vi "Compile and Export Settings.vi"(8 "error in (no error)":errorcluster, 11 "Device Item Ref in":T1 format="%.0x") -> (0 "error out":errorcluster)   [LabVIEW 2015, in "Protection and Counter Addon System Explorer.lvlib"]
uses:
  Protection and Counter Addon System Explorer.lvlib
  <vilib>/NI Veristand/Custom Device API/Custom Device Item Ref.ctl
  Shared/Types/Exported.OnCompile.ctl
  Shared/Types/XNET Settings.ctl
  SubModules/Frame Protection Support/Source/Shared/Types/Exported Frame Settings.ctl
  SubModules/Frame Protection Support/Source/Shared/Types/Exported Frame Type.ctl
  SubModules/Frame Protection Support/Source/Shared/Types/Exported Protection Settings.ctl
  SubModules/Frame Protection Support/Source/Shared/Types/Protection Type.ctl
  SubModules/Frame Protection Support/Source/Shared/Types/XNET Signal Configuration.ctl
  SubModules/Frame Protection Support/Source/Shared/Types/Exported Counter Settings.ctl
  SubModules/Frame Protection Support/Source/Shared/Types/Exported Event Trigger Type.ctl
  Shared/Types/986x.ctl
  <vilib>/NI Veristand/Custom Device Tools/Custom Device Utility Library/Search Direction.ctl
  SubModules/Frame Protection Support/Source/System Explorer/Types/Export Frame GUIDs List.ctl
  SubModules/Frame Protection Support/Source/System Explorer/Types/Export Frames List and Type.ctl
  SubModules/Frame Protection Support/Source/System Explorer/Types/Exported Frame Settings.ctl
  Shared/SubVIs/GUID Lookup.vi
  <vilib>/NI Veristand/Custom Device API/NI VeriStand - Get Item Property.vi
  <vilib>/NI Veristand/Custom Device API/Get Item Property (Boolean).vi
  <vilib>/NI Veristand/Custom Device API/Get Item Property (String).vi
  FileDependency.Get.Target Path.vi
  <vilib>/NI Veristand/Custom Device Tools/Custom Device Utility Library/NI VeriStand - Search for Item by GUID.vi
  <vilib>/NI Veristand/Custom Device API/Set Item Property (Variant).vi
  <vilib>/NI VeriStand/Custom Device Tools/Custom Device Utility Library/Custom Device Utility Library.lvlib
  Shared/Protection and Counter Addon Shared.lvlib
  <vilib>/NI VeriStand/Custom Device API/Custom Device API.lvlib
  SubModules/Frame Protection Support/Source/Shared/Protection and Counter Support Shared.lvlib
  <vilib>/NI/NIVS Inline Async API/_Data Access System Explorer/Data Access System Explorer.lvlib
  SubModules/Frame Protection Support/Source/System Explorer/Protection and Counter Support System Explorer.lvlib
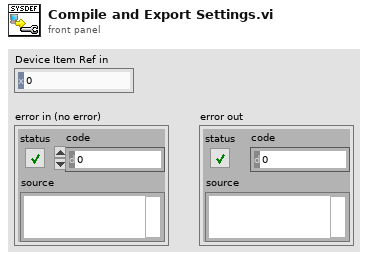
[diagram p1: front panel]
types:
  T1 = typedef "Custom Device API.lvlib/Custom Device Item Ref.ctl" = u64
  T2 = typedef "Protection and Counter Support System Explorer.lvlib/Export Frame GUIDs List.ctl" = cluster{"Signal Page GUID":string, "Rolling Counter Value GUID":string, "Protection Value GUID":string}
  T3 = typedef "Protection and Counter Support Shared.lvlib/Exported Frame Type.ctl" = enum16{"Periodic", "Event", "Periodic/Event"}
  T4 = typedef "Custom Device Utility Library.lvlib/Search Direction.ctl" = enum16{"Down", "Up"}
  T5 = cluster{"Name":string, "Type":enum16{"Output/Write", "Input/Read", "Input/ReadWrite"}, "VS Refs":T1[]}
  T6 = typedef "Protection and Counter Addon Shared.lvlib/Exported.OnCompile.ctl" = cluster{"XNET Settings":T7, "Frames":T8[], "986x Support":T14}
  T7 = typedef "Protection and Counter Addon Shared.lvlib/XNET Settings.ctl" = cluster{"Database":refnum<k21>, "Cluster":refnum<k21>, "Port":string, "Baud rate [Bd]":u64, "Termination":u32, "CAN I/O Mode":u32, "FD Baud rate [Bd]":u64, "Priority":i32, "Use Legacy":bool}
  T8 = typedef "Protection and Counter Support Shared.lvlib/Exported Frame Settings.ctl" = cluster{"Type":T3, "Frame ID":u32, "Payload Length":u32, "Signal XNET Paths":string[], "Frame.PrevData":dbl[], "VS Offset":i32, "VS Length":i32, "Generation Period":u32, "Has Protection?":bool, "Protection Configurations":T9[], "Has Counter":bool, "Counter Configurations":T12[], "Has Disable?":bool, "Disable VS Index":i32, "Transmit Trigger":T13, "Trigger VS Index":i32}
  T9 = typedef "Protection and Counter Support Shared.lvlib/Exported Protection Settings.ctl" = cluster{"Protection Frame Index":i32, "Protection Type":T10, "Data Indeces":i32[], "Initialized Data Array":dbl[], "Protection Signal XNET Paths":string[], "CRC Channels":T11[], "Protection VS Update Index":i32}
  T10 = typedef "Protection and Counter Support Shared.lvlib/Protection Type.ctl" = enum16{"Arb ID + Bytes Checksum with Inversion", "Arb ID + Bytes CRC with Inversion", "Reversed Raw Signal Checksum with Inversion"}
  T11 = typedef "Protection and Counter Support Shared.lvlib/XNET Signal Configuration.ctl" = cluster{"Start Bit":i32, "Name":string, "Number of bits":i32, "Scale":dbl, "Offset":dbl, "Data Type":u32}
  T12 = typedef "Protection and Counter Support Shared.lvlib/Exported Counter Settings.ctl" = cluster{"Counter Frame Index":i32, "Max Count":dbl, "Counter VS Index":i32}
  T13 = typedef "Protection and Counter Support Shared.lvlib/Exported Event Trigger Type.ctl" = enum16{"Channel value change", "Trigger channel (not zero)", "Channel value change or trigger channel (not zero)", "Trigger channel (any value change)", "Channel value change or trigger channel (any value change)"}
  T14 = typedef "Protection and Counter Addon Shared.lvlib/986x.ctl" = cluster{"Enable":bool, "RIO Device":string, "Bitfile":path}
  T15 = typedef "Protection and Counter Support System Explorer.lvlib/Export Frames List and Type.ctl" = cluster{"Type":T3, "Frame Refs":T1[], "Frame Settings":T16[]}
  T16 = typedef "Protection and Counter Support System Explorer.lvlib/Exported Frame Settings.ctl" = cluster{"ID":u32, "Disable Transmission":bool, "Disable Transmission Ref":T1, "Transmit Trigger":T13, "Transmit Trigger Ref":T1}
  T17 = typedef "Protection and Counter Addon System Explorer.lvlib/Frame Settings.ctl" = cluster{"ID":u32, "Disable Transmission":bool, "Disable Transmission Ref":T1, "Transmit Trigger":T18, "Transmit Trigger Ref":T1}
  T18 = typedef "Protection and Counter Addon System Explorer.lvlib/Event Trigger Type.ctl" = enum16{"Channel value change", "Trigger channel (not zero)", "Channel value change or trigger channel (not zero)", "Trigger channel (any value change)", "Channel value change or trigger channel (any value change)"}
  T19 = cluster{"Name":string, "Type":enum16{"Output/Write", "Input/Read", "Input/ReadWrite"}, "VS Refs":T1[]}[]
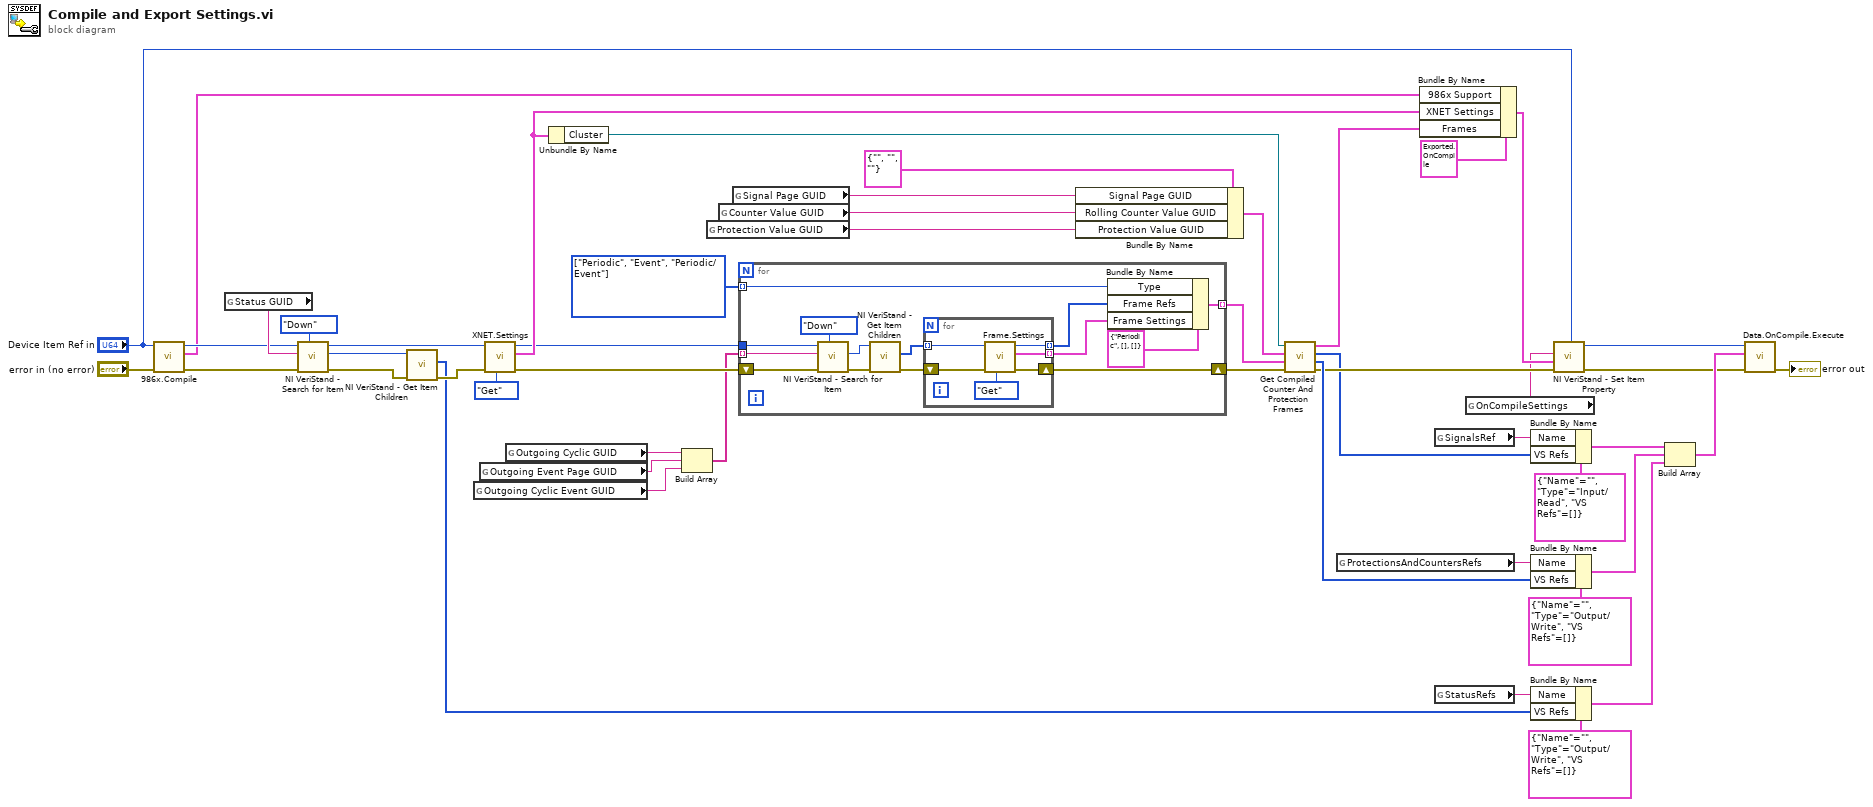
[diagram p0: block diagram]
diagram:
  w13 = T3[] [enum."Periodic", enum."Event", enum."Periodic/Event"] items=["Periodic", "Event", "Periodic/Event"]
  n1 = call "986x.Compile.vi"("error in (no error)"="error in (no error)", "Item Ref in"="Device Item Ref in") -> ("error out"=w21:errorcluster, "986x Support"=w10:T14, "Item Ref out"=w20:T1)  [unwired: 7 in]
  n2 = global read "GUID Lookup.vi" "Status GUID"() -> (w29:string)
  n3 = call-poly <vilib>:"NI VeriStand - Search for Item.vi"("Direction (Down)"=Search_Direction."Down", "error in"=w21, "Item GUID"=w29, "Section Ref in"=w20) -> ("error out"=w26:errorcluster, "Item Ref"=w27:T1, "Section Ref out"=w28:T1)  [unwired: 4 in, 1 out]
  n4 = call <vilib>:"NI VeriStand - Get Item Children.vi"("error in (no error)"=w26, "Item Ref in"=w27) -> ("error out"=w25:errorcluster, "Child Refs"=w24:T1[])  [unwired: 6 in, 2 out]
  n5 = global read "GUID Lookup.vi" "Outgoing Cyclic Event GUID"() -> (w4:string)
  n6 = global read "GUID Lookup.vi" "Outgoing Event Page GUID"() -> (w5:string)
  n7 = call "XNET.Settings.vi"("Action"=enum8{"Get", "Set"}."Get", "error in (no error)"=w25, "Parent Ref in"=w28) -> ("error out"=w3:errorcluster, "XNET Settings"=w46:T7, "Item Ref out"=w2:T1)  [unwired: 6 in]
  n8 = global read "GUID Lookup.vi" "Outgoing Cyclic GUID"() -> (w6:string)
  n9 = Unbundle By Name(w46) -> ("Cluster"=w48:refnum<k21>)
  n10 = Build Array(w6, w5, w4) -> (w1:string[])
  n11 = global read "GUID Lookup.vi" "Protection Value GUID"() -> (w17:string)
  n12 = global read "GUID Lookup.vi" "Counter Value GUID"() -> (w18:string)
  n13 = global read "GUID Lookup.vi" "Signal Page GUID"() -> (w19:string)
  n14 = for {
    shift-right: [w50] -> w14
    shift-left: w3 -> [w60]
    tunnel: w13 -> [w63] mode=indexing
    tunnel: [w62] -> w12 mode=indexing
    tunnel: w2 -> [w59]
    tunnel: w1 -> [w58] mode=indexing
    n15 = call-poly <vilib>:"NI VeriStand - Search for Item.vi"("Direction (Down)"=Search_Direction."Down", "error in"=w60, "Item GUID"=w58, "Section Ref in"=w59) -> ("error out"=w56:errorcluster, "Item Ref"=w57:T1)  [unwired: 4 in, 2 out]
    n16 = call <vilib>:"NI VeriStand - Get Item Children.vi"("error in (no error)"=w56, "Item Ref in"=w57) -> ("error out"=w54:errorcluster, "Child Refs"=w53:T1[])  [unwired: 6 in, 2 out]
    n17 = for {
      tunnel: w53 -> [w67] mode=indexing
      shift-right: [w66] -> w50
      shift-left: w54 -> [w68]
      tunnel: [w65] -> w52 mode=indexing
      tunnel: [w64] -> w51 mode=indexing
      n18 = call "Frame.Settings.vi"("Action"=enum8{"Get", "Set"}."Get", "error in (no error)"=w68, "Item Ref in"=w67) -> ("error out"=w66:errorcluster, "Frame.Settings"=w64:T17, "Item Ref out"=w65:T1)  [unwired: 6 in]
    }
    n19 = Bundle By Name(cluster=T15 {"Type"=enum."Periodic", "Frame Refs"=[], "Frame Settings"=[]} ("Export Frames List and Type"), "Type"=w63, "Frame Refs"=w52, "Frame Settings"=w51) -> (w62:T15)
  }
  n20 = Bundle By Name(cluster=T2 {"Signal Page GUID"="", "Rolling Counter Value GUID"="", "Protection Value GUID"=""}, "Signal Page GUID"=w19, "Rolling Counter Value GUID"=w18, "Protection Value GUID"=w17) -> (w15:T2)
  n21 = call "Get Compiled Counter And Protection Frames.vi"("error in (no error)"=w14, "Frames per type"=w12, "GUIDs"=w15, "XNET Cluster"=w48) -> ("error out"=w39:errorcluster, "Counters and Protection Refs"=w40:T1[], "Signals Refs"=w9:T1[], "Frames"=w8:T8[])  [unwired: 4 in]
  n22 = global read "GUID Lookup.vi" "ProtectionsAndCountersRefs"() -> (w35:string)
  n23 = Bundle By Name(cluster=T6 {"XNET Settings"={"Database"="", "Cluster"="", "Port"="", "Baud rate [Bd]"=500000, "Termination"=1, "CAN I/O Mode"=0, "FD Baud rate [Bd]"=500000, "Priority"=100, "Use Legacy"=FALSE}, "Frames"=[], "986x Support"={"Enable"=FALSE, "RIO Device"="", "Bitfile"=path ""}}, "986x Support"=w10, "XNET Settings"=w46, "Frames"=w8) -> (w45:T6)
  n24 = global read "GUID Lookup.vi" "SignalsRef"() -> (w36:string)
  n25 = global read "GUID Lookup.vi" "StatusRefs"() -> (w31:string)
  n26 = global read "GUID Lookup.vi" "OnCompileSettings"() -> (w34:string)
  n27 = Bundle By Name(cluster=T5 {"Name"="", "Type"=enum."Input/Read", "VS Refs"=[]} ("Group"), "Name"=w36, "VS Refs"=w9) -> (w43:T5)
  n28 = Bundle By Name(cluster=T5 {"Name"="", "Type"=enum."Output/Write", "VS Refs"=[]} ("Group"), "Name"=w35, "VS Refs"=w40) -> (w33:T5)
  n29 = Bundle By Name(cluster=T5 {"Name"="", "Type"=enum."Output/Write", "VS Refs"=[]} ("Group"), "Name"=w31, "VS Refs"=w24) -> (w11:T5)
  n30 = call-poly <vilib>:"NI VeriStand - Set Item Property.vi"("error in (no error)"=w39, "Value"=w45, "Property Name"=w34, "Item Ref in"="Device Item Ref in") -> ("error out"=w38:errorcluster, "Item Ref out"=w37:T1)  [unwired: 5 in, 1 out]
  n31 = Build Array(w43, w33, w11) -> (w42:T19)
  n32 = call <vilib>:"Data.OnCompile.Execute.vi"("error in"=w38, "VS Ref Groups"=w42, "Custom Device Ref"=w37) -> ("error out"=→"error out":errorcluster)  [unwired: 7 in, 1 out]
